vi "ControllerGUI.vi"() -> ()   [LabVIEW 2024]
panel:
  out "91io":picture
  out "51screen":picture
  out "81wind":picture
  in  "Save":bool
  in  "Save File":path
  in  "Load":bool
  in  "Read Config":path
  in  "Mode 4":bool
  in  "Mode 3":bool
  in  "Mode 2":bool
  in  "Mode 1":bool
  out "105led":picture
  out "background":picture
  # "Sandbox Monitor"
  # "Will be replaced by individual status display"
  # "Save data (in the furture)"
  # "Sandbox Control"
  # "Predefined modes"
  # "Load user-defined config"
  # "Right click to open menu"
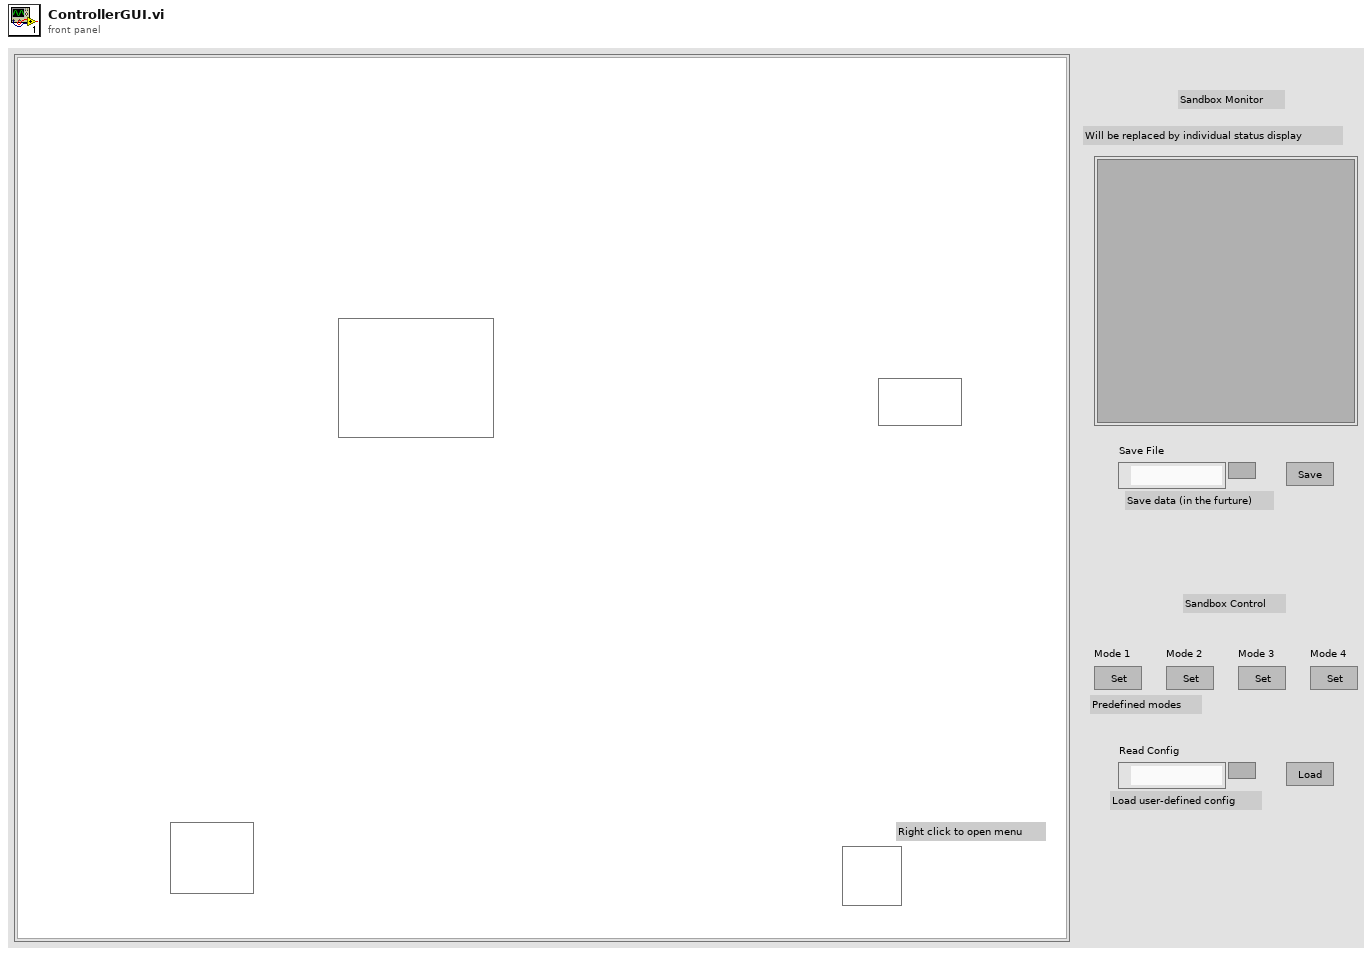
[diagram p1: front panel]
types:
  T1 = typedef "imagedata.ctl" = cluster{"image type":i32, "image depth":i32, "image":u8[], "mask":u8[], "colors":u32[], "Rectangle":cluster{"left":i16, "top":i16, "right":i16, "bottom":i16}}
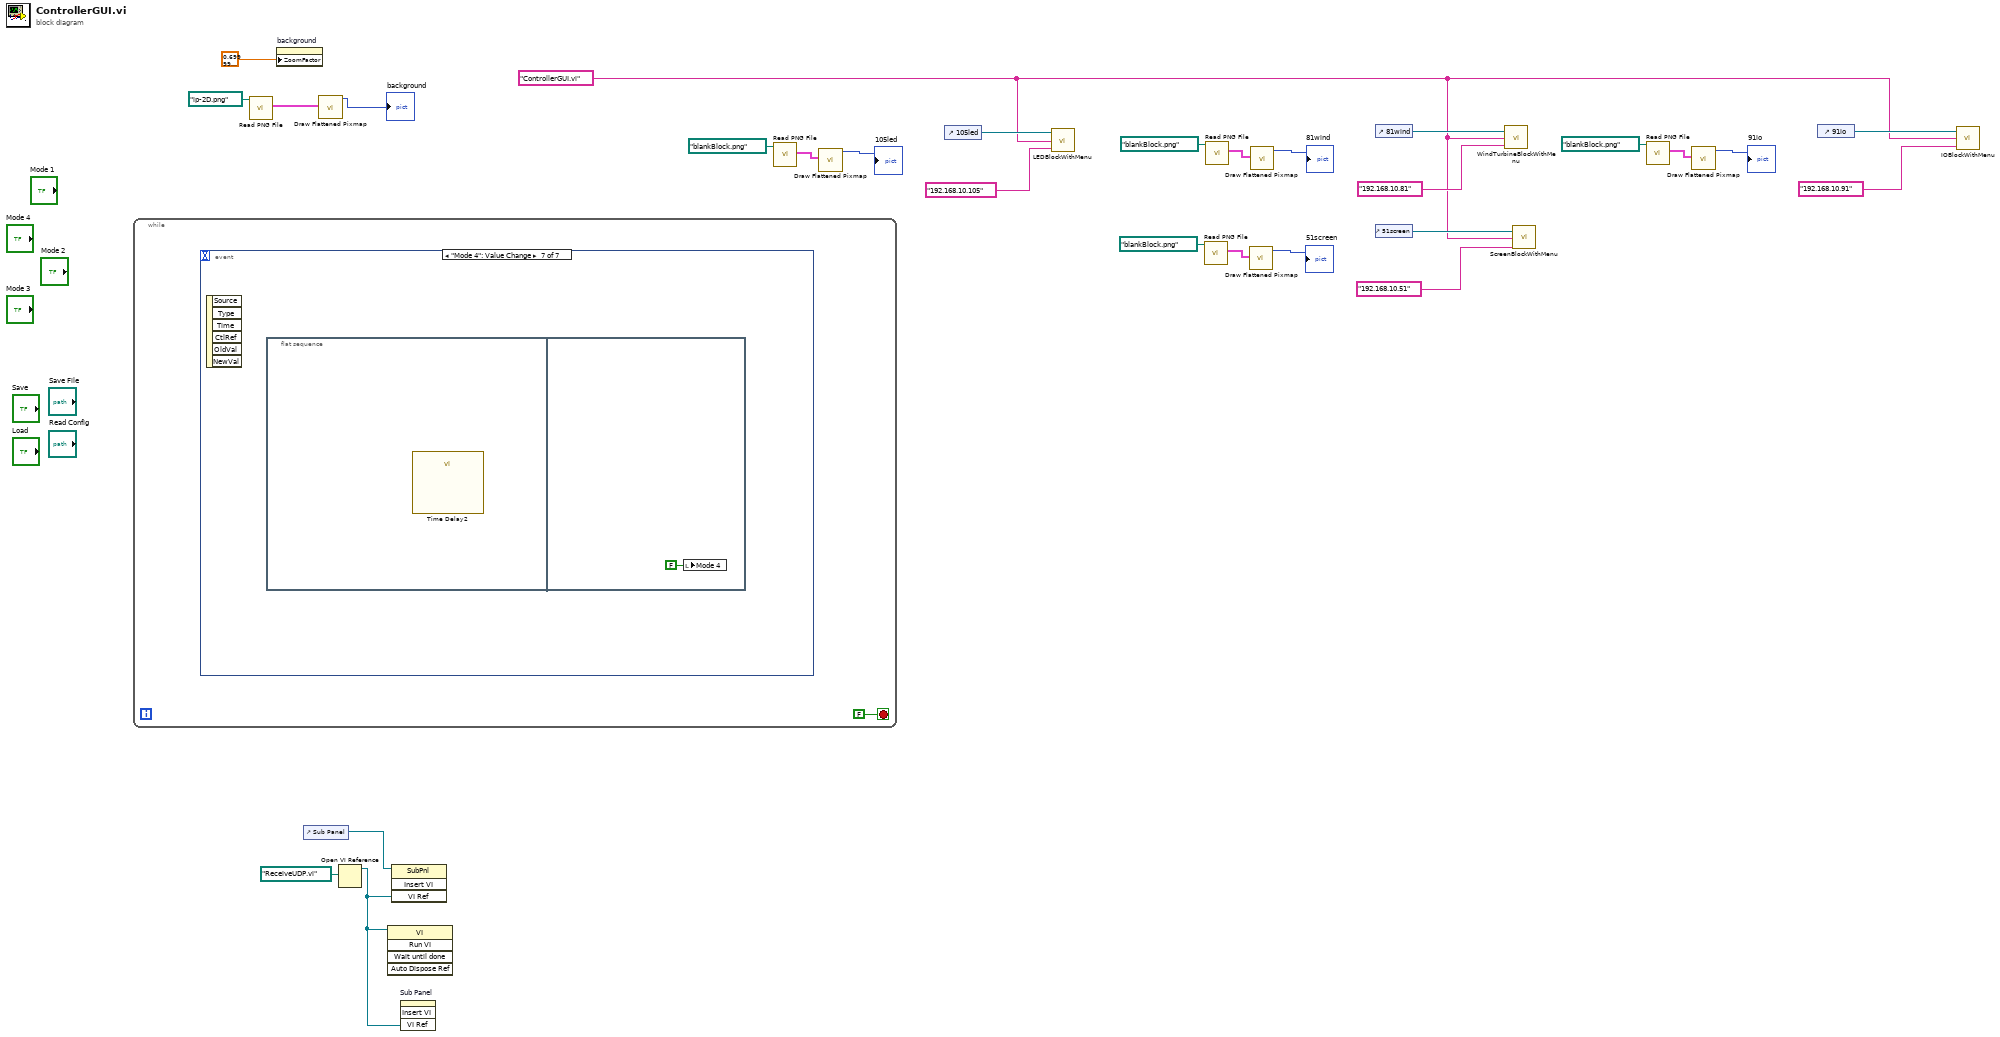
[diagram p0: block diagram]
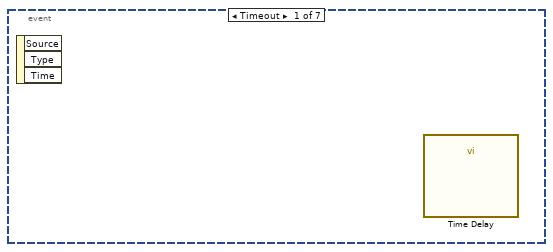
[diagram p2: hidden frame]
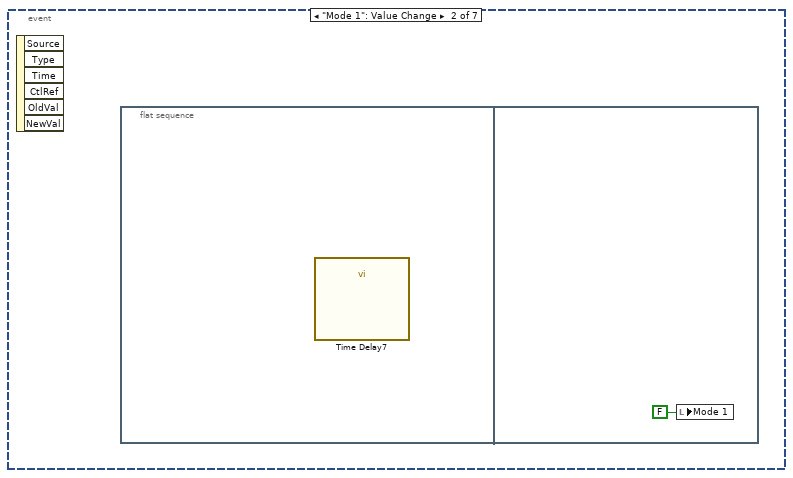
[diagram p3: hidden frame]
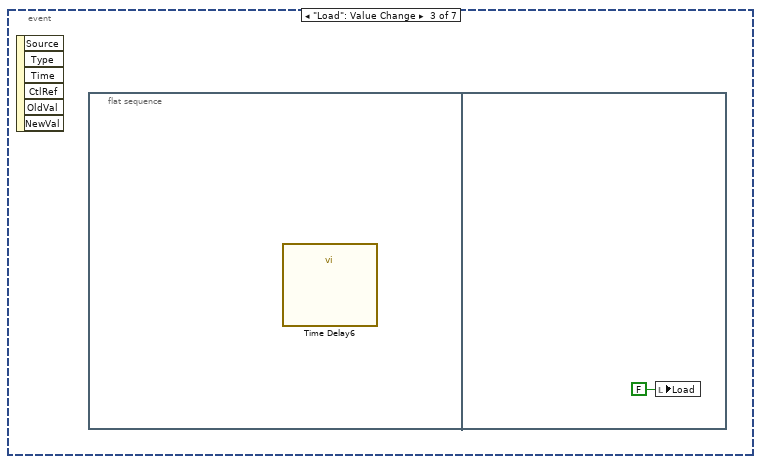
[diagram p4: hidden frame]
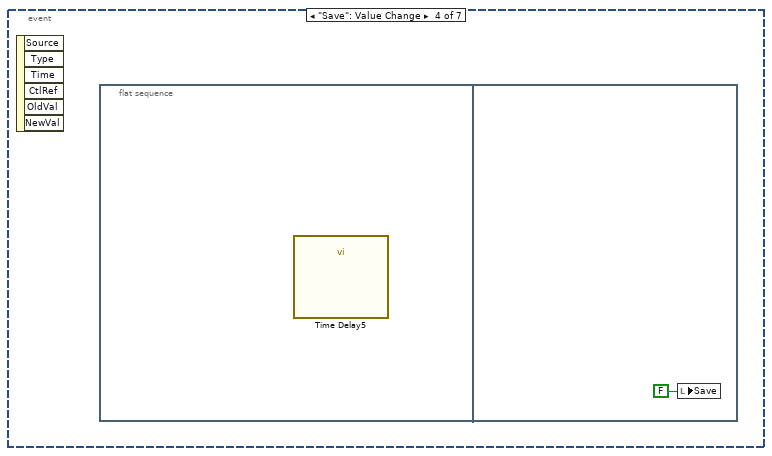
[diagram p5: hidden frame]
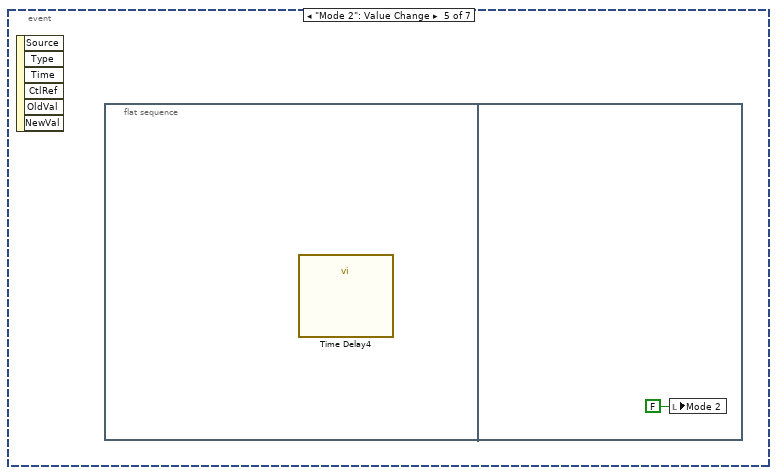
[diagram p6: hidden frame]
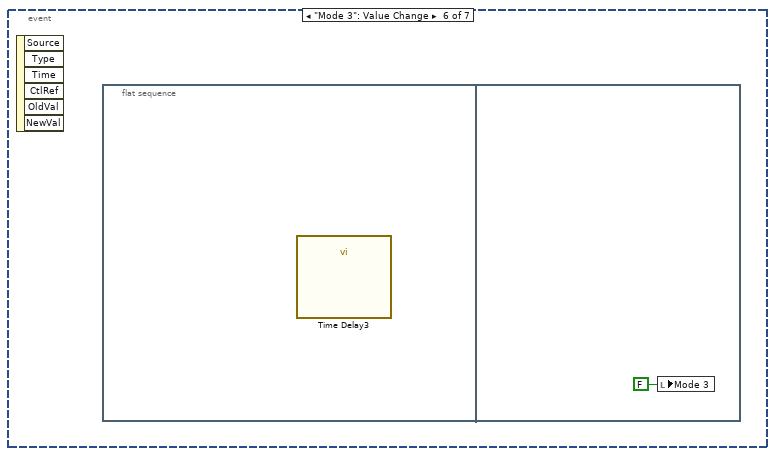
[diagram p7: hidden frame]
diagram:
  w6 = "ControllerGUI.vi"
  n1 = while {
    stop <- FALSE stop-if-true
    n2 = event shown="[6] \"Mode 4\": Value Change" {
      selector: _ -> [_ _ _ _ _ _ _]
      dyn-events: _ -> [_ _ _ _ _ _ _]
      timeout: _ -> [_ _ _ _ _ _ _]
      event Timeout {
        n3 = event-data() -> ()  [unwired: 1 in, 3 out]
        n4 = call "Time Delay"() -> ()  [unwired: 11 in, 1 out]
      }
      event "Mode 1": Value Change {
        n5 = event-data() -> ()  [unwired: 1 in, 6 out]
        n6 = flat-sequence {
          frame #0 {
            n7 = call "Time Delay7"() -> ()  [unwired: 11 in, 1 out]
          }
          frame #1 {
            n8 = local write "Mode 1"(FALSE ("Mode 1")) -> ()
          }
        }
      }
      event "Load": Value Change {
        n9 = event-data() -> ()  [unwired: 1 in, 6 out]
        n10 = flat-sequence {
          frame #0 {
            n11 = call "Time Delay6"() -> ()  [unwired: 11 in, 1 out]
          }
          frame #1 {
            n12 = local write "Load"(FALSE ("Load")) -> ()
          }
        }
      }
      event "Save": Value Change {
        n13 = event-data() -> ()  [unwired: 1 in, 6 out]
        n14 = flat-sequence {
          frame #0 {
            n15 = call "Time Delay5"() -> ()  [unwired: 11 in, 1 out]
          }
          frame #1 {
            n16 = local write "Save"(FALSE ("Save")) -> ()
          }
        }
      }
      event "Mode 2": Value Change {
        n17 = event-data() -> ()  [unwired: 1 in, 6 out]
        n18 = flat-sequence {
          frame #0 {
            n19 = call "Time Delay4"() -> ()  [unwired: 11 in, 1 out]
          }
          frame #1 {
            n20 = local write "Mode 2"(FALSE ("Mode 2")) -> ()
          }
        }
      }
      event "Mode 3": Value Change {
        n21 = event-data() -> ()  [unwired: 1 in, 6 out]
        n22 = flat-sequence {
          frame #0 {
            n23 = call "Time Delay3"() -> ()  [unwired: 11 in, 1 out]
          }
          frame #1 {
            n24 = local write "Mode 3"(FALSE ("Mode 3")) -> ()
          }
        }
      }
      event "Mode 4": Value Change {
        n25 = event-data() -> ()  [unwired: 1 in, 6 out]
        n26 = flat-sequence {
          frame #0 {
            n27 = call "Time Delay2"() -> ()  [unwired: 11 in, 1 out]
          }
          frame #1 {
            n28 = local write "Mode 4"(FALSE ("Mode 4")) -> ()
          }
        }
      }
    }
  }
  n29 = call <vilib>:"Read PNG File.vi"("path to PNG file"=path "ip-2D.png") -> ("image data"=w28:T1)  [unwired: 8 in, 2 out]
  n30 = property on="background" class="Pict"("ZoomFactor"=sgl 0.7 ("Zoom Factor")) -> ()  [unwired: 2 in, 2 out]
  n31 = control-ref of="Sub Panel"() -> (w1:refnum<vi>)
  n32 = call <vilib>:"Draw Flattened Pixmap.vi"("image data"=w28) -> ("new picture"=→"background":picture)  [unwired: 8 in]
  n33 = Open VI Reference(vi path=path "ReceiveUDP.vi") -> (vi reference=w2:refnum<vi>)  [unwired: 5 in, 1 out]
  n34 = invoke class="VI" method="Run VI"(reference=w2) -> ()  [unwired: 4 in, 5 out]
  n35 = invoke class="SubPnl" method="Insert VI"(reference=w1, "VI Ref"=w2) -> ()  [unwired: 2 in, 4 out]
  n36 = invoke on="Sub Panel" class="SubPnl" method="Insert VI"("VI Ref"=w2) -> ()  [unwired: 3 in, 4 out]
  n37 = call <vilib>:"Read PNG File.vi"("path to PNG file"=path "blankBlock.png") -> ("image data"=w24:T1)  [unwired: 8 in, 2 out]
  n38 = call <vilib>:"Draw Flattened Pixmap.vi"("image data"=w24) -> ("new picture"=→"105led":picture)  [unwired: 8 in]
  n39 = control-ref of="105led"() -> (w22:refnum<vi>)
  n40 = call "LEDBlockWithMenu.vi"("IP"="192.168.10.105", "Main GUI Path"=w6, "Ctl Refnum"=w22) -> ()
  n41 = call <vilib>:"Read PNG File.vi"("path to PNG file"=path "blankBlock.png") -> ("image data"=w14:T1)  [unwired: 8 in, 2 out]
  n42 = call <vilib>:"Read PNG File.vi"("path to PNG file"=path "blankBlock.png") -> ("image data"=w19:T1)  [unwired: 8 in, 2 out]
  n43 = call <vilib>:"Draw Flattened Pixmap.vi"("image data"=w14) -> ("new picture"=→"51screen":picture)  [unwired: 8 in]
  n44 = call <vilib>:"Draw Flattened Pixmap.vi"("image data"=w19) -> ("new picture"=→"81wind":picture)  [unwired: 8 in]
  n45 = control-ref of="51screen"() -> (w12:refnum<vi>)
  n46 = control-ref of="81wind"() -> (w17:refnum<vi>)
  n47 = call "WindTurbineBlockWithMenu.vi"("IP"="192.168.10.81", "Main GUI Path"=w6, "Ctl Refnum"=w17) -> ()
  n48 = call "ScreenBlockWithMenu.vi"("IP"="192.168.10.51", "Main GUI Path"=w6, "Ctl Refnum"=w12) -> ()
  n49 = call <vilib>:"Read PNG File.vi"("path to PNG file"=path "blankBlock.png") -> ("image data"=w9:T1)  [unwired: 8 in, 2 out]
  n50 = call <vilib>:"Draw Flattened Pixmap.vi"("image data"=w9) -> ("new picture"=→"91io":picture)  [unwired: 8 in]
  n51 = control-ref of="91io"() -> (w7:refnum<vi>)
  n52 = call "IOBlockWithMenu.vi"("IP"="192.168.10.91", "Main GUI Path"=w6, "Ctl Refnum"=w7) -> ()
